vi "Runtime Test.vi"() -> (0 "final error":errorcluster, 1 "correct execution settings":bool, 2 "Pass Input":bool, 3 "Pass Output":bool)   [LabVIEW 2015, in "SystemLink Tag Module tests.lvlib"]
doc: "This VI shows an example for how to test the Runtime functionality of the module. This will need to be modified according to module functionality."
uses:
  SystemLink Tag Module tests.lvlib
  module/execution/SystemLink runtime.lvclass
  module/configuration/SystemLink configuration.lvclass
panel:
  out "Names":string[](array[string])
  out "init error":errorcluster
  out "invalid configuration":errorcluster
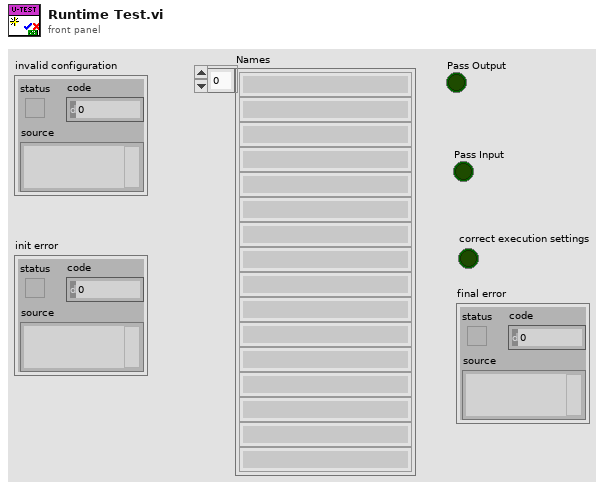
[diagram p1: front panel]
types:
  T1 = typedef "TBM channel.lvclass/data tables.ctl" = cluster{"input data":T2, "processing parameter":T2, "processing result":T2, "output data":T2}
  T2 = typedef "tag bus.lvlib/dictionary table pair.ctl" = cluster{"data dictionary":refnum<class "data dictionary.lvclass">, "data table":T3}
  T3 = typedef "tag bus.lvlib/data table.lvlib/data table.ctl" = cluster{"Double":dbl[], "Single":sgl[], "I64":i64[], "I32":i32[], "I16":i16[], "I8":i8[], "U64":u64[], "U32":u32[], "U16":u16[], "U8":u8[], "Boolean":bool[], "String":string[], "Array of Double":cluster{"DBL Array":dbl[]}[], "Array of Single":cluster{"SGL Array":sgl[]}[], "Array of I64":cluster{"I64 Array":i64[]}[], "Array of I32":cluster{"I32 Array":i32[]}[], "Array of I16":cluster{"I16 Array":i16[]}[], "Array of I8":cluster{"I8 Array":i8[]}[], "Array of U64":cluster{"U64 Array":u64[]}[], "Array of U32":cluster{"U32 Array":u32[]}[], "Array of U16":cluster{"U16 Array":u16[]}[], "Array of U8":cluster{"U8 Array":u8[]}[], "Array of Boolean":cluster{"Boolean Array":bool[]}[], "Array of String":cluster{"String Array":string[]}[]}
  T4 = typedef "TBM module execution interface.lvclass/execution settings.ctl" = cluster{"reads inputs":bool, "processes data":bool, "writes outputs":bool}
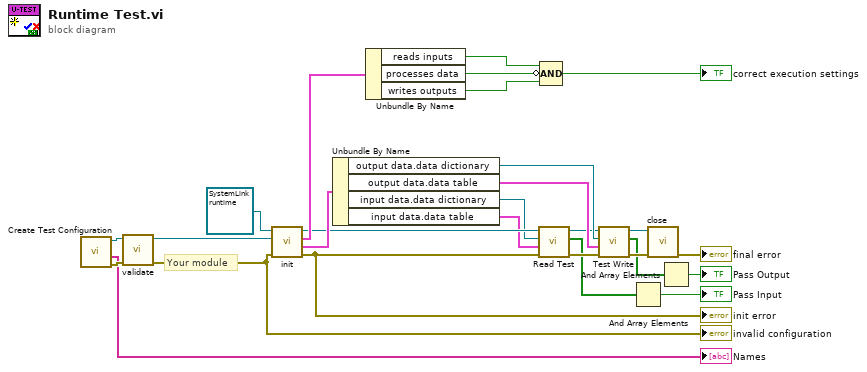
[diagram p0: block diagram]
diagram:
  # "Your module"
  n1 = call "Create Test Configuration.vi"() -> ("error out"=w8:errorcluster, "Names"=→"Names":string[], "Module Configuration"=w9:refnum<class "SystemLink configuration.lvclass">)  [unwired: 6 in, 3 out]
  n2 = call-dynamic "validate.vi"("error in"=w8, "SystemLin Tag Module configuration in"=w9) -> ("error out"=w26:errorcluster, "SystemLin Tag Module configuration out"=w27:refnum<class "SystemLink configuration.lvclass">)  [unwired: 8 in]
  "invalid configuration" <- w26
  n3 = call-dynamic "init.vi"("error in"=w26, "TBM module configuration in"=w27, "SystemLin Tag Module runtime in"=refnum<class "SystemLink runtime.lvclass"> refnum ("tag bus configurable plugin module")) -> ("error out"=w18:errorcluster, "data allocations"=w19:T1, "execution settings"=w24:T4, "SystemLin Tag Module runtime out"=w17:refnum<class "SystemLink runtime.lvclass">)  [unwired: 5 in]
  "init error" <- w18
  n4 = Unbundle By Name(w19) -> ("output data.data dictionary"=w16:refnum<class "data dictionary.lvclass">, "output data.data table"=w15:T3, "input data.data dictionary"=w3:refnum<class "data dictionary.lvclass">, "input data.data table"=w4:T3)
  n5 = Unbundle By Name(w24) -> ("reads inputs"=w21:bool, "processes data"=w23:bool, "writes outputs"=w22:bool)
  n6 = call "Read Test.vi"("error in (no error)"=w18, "data table"=w4, "data dictionary"=w3, "runtime in"=w17) -> ("error out"=w14:errorcluster, "Pass"=w5:bool[], "runtime out"=w13:refnum<class "SystemLink runtime.lvclass">)  [unwired: 5 in]
  n7 = Compound Arithmetic op=AND(w21, invert w23, w22) -> (→"correct execution settings":bool)
  n8 = call "Test Write.vi"("error in (no error)"=w14, "data table"=w15, "data dictionary"=w16, "runtime in"=w13) -> ("error out"=w11:errorcluster, "Pass"=w6:bool[], "runtime out"=w12:refnum<class "SystemLink runtime.lvclass">)  [unwired: 5 in]
  n9 = And Array Elements(Boolean array=w5) -> (logical AND=→"Pass Input":bool)
  n10 = call-dynamic "close.vi"("error in"=w11, "SystemLin Tag Module runtime in"=w12) -> ("error out"=→"final error":errorcluster)  [unwired: 9 in]
  n11 = And Array Elements(Boolean array=w6) -> (logical AND=→"Pass Output":bool)
